vi "ArmPathPlanner.vi"(0 "StartPoint":T5, 1 "EndPoint":T5, 2 "PathPointSpacing (in)":dbl=0.25, 3 "MinArmLength":dbl=44.0, 4 "MaxArmLength":dbl=68.0, 5 "AvoidancePolygon":T4, 7 "MotionProfileGeneratorParameters":T3={"Trajectory Point Interval (ms)"=10, "Maximum Travel Speed (units/s)"=0.0, "Velocity Ramp Time (ms)"=0.0, "Acceleration Ramp Time (ms)"=1.0} {"Acceleration Ramp Time (ms)" min=1.0; "Velocity Ramp Time (ms)" min=1.0; "Maximum Travel Speed (units/s)" min=0.0; "Trajectory Point Interval (ms)" items=["TrajectoryDuration_0ms"=0, "TrajectoryDuration_5ms"=5, "TrajectoryDuration_10ms"=10, "TrajectoryDuration_20ms"=20, "TrajectoryDuration_30ms"=30, "TrajectoryDuration_40ms"=40, "TrajectoryDuration_50ms"=50, "TrajectoryDuration_100ms"=100]}) -> (14 "Path":T6[](array[typedef]), 15 "RotatePath":T1[](array[typedef]) {"Time (ms)" items=["TrajectoryDuration_0ms"=0, "TrajectoryDuration_5ms"=5, "TrajectoryDuration_10ms"=10, "TrajectoryDuration_20ms"=20, "TrajectoryDuration_30ms"=30, "TrajectoryDuration_40ms"=40, "TrajectoryDuration_50ms"=50, "TrajectoryDuration_100ms"=100]}, 16 "ExtendPath":T1[](array[typedef]) {"Time (ms)" items=["TrajectoryDuration_0ms"=0, "TrajectoryDuration_5ms"=5, "TrajectoryDuration_10ms"=10, "TrajectoryDuration_20ms"=20, "TrajectoryDuration_30ms"=30, "TrajectoryDuration_40ms"=40, "TrajectoryDuration_50ms"=50, "TrajectoryDuration_100ms"=100]}, 19 "PathLength (in)":dbl)   [LabVIEW 2017]
uses:
  TypeDefs/ArmCoordinate.ctl
  ArgosLib/Path Planning/TypeDefs/Point2D.ctl
  ArgosLib/Path Planning/TypeDefs/Polygon2D.ctl
  General/MotionProfiling/TypeDefs/MotionProfileGeneratorParams.ctl
  <vilib>/Rock Robotics/WPI/ThirdParty/Phoenix-LabVIEW/Motor Controller/Controls/CTRE_Phoenix_MotorControl_TrajectoryPointTimeDur.ctl
  General/MotionProfiling/TypeDefs/TrajectoryPoint.ctl
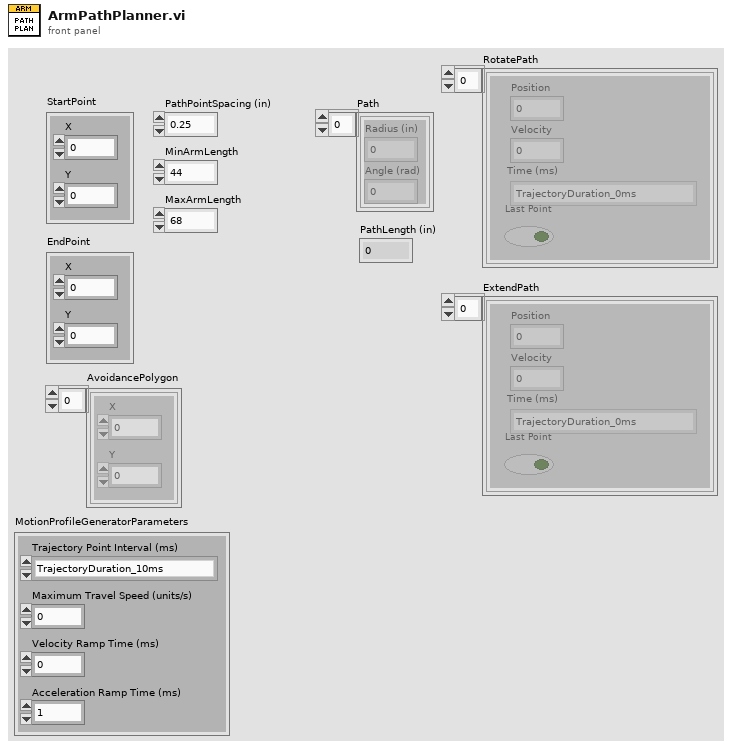
[diagram p1: front panel]
types:
  T1 = typedef "TrajectoryPoint.ctl" = cluster{"Position ":dbl, "Velocity ":dbl, "Time (ms)":T2, "Last Point":bool}
  T2 = typedef "CTRE_Phoenix_MotorControl_TrajectoryPointTimeDur.ctl" = i32
  T3 = typedef "MotionProfileGeneratorParams.ctl" = cluster{"Trajectory Point Interval (ms)":T2, "Maximum Travel Speed (units/s)":dbl, "Velocity Ramp Time (ms)":dbl, "Acceleration Ramp Time (ms)":dbl}
  T4 = typedef "Polygon2D.ctl" = T5[]
  T5 = typedef "Point2D.ctl" = cluster{"X":dbl, "Y":dbl}
  T6 = typedef "ArmCoordinate.ctl" = cluster{"Radius (in)":dbl, "Angle (rad)":dbl}
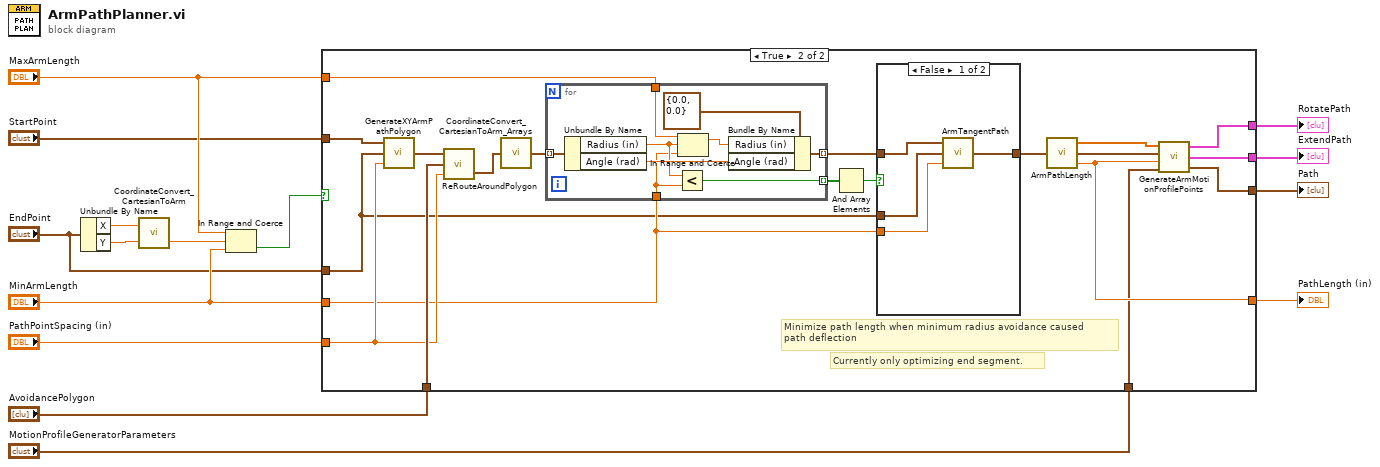
[diagram p0: block diagram]
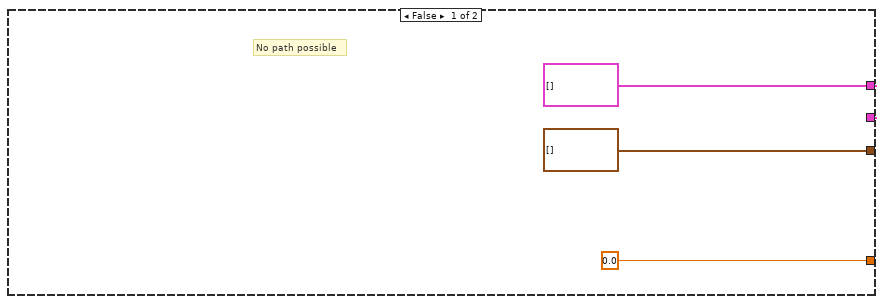
[diagram p2: hidden frame]
diagram:
  n1 = Unbundle By Name("EndPoint") -> ("X"=w8:dbl, "Y"=w7:dbl)
  n2 = call "CoordinateConvert_CartesianToArm.vi"("Y (in)"=w7, "X (in)"=w8) -> ("Radius (in)"=w15:dbl)  [unwired: 1 out]
  n3 = In Range and Coerce(upper limit="MaxArmLength", x=w15, lower limit="MinArmLength") -> (In Range?=w14:bool)  [unwired: 1 out]
  n4 = case shown="True" w14 {
    tunnel: [T6[] [] ("ArmPathOut") w27] -> w9
    tunnel: [0.0 w29] -> w13
    tunnel: "MinArmLength" -> [_ w20]
    tunnel: "MaxArmLength" -> [_ w38]
    tunnel: "PathPointSpacing (in)" -> [_ w33]
    tunnel: "StartPoint" -> [_ w37]
    tunnel: "EndPoint" -> [_ w19]
    tunnel: "AvoidancePolygon" -> [_ w34]
    tunnel: "MotionProfileGeneratorParameters" -> [_ w28]
    tunnel: [w16 w26] -> w2
    tunnel: [w16 w25] -> w1
    frame False {
      w16 = T1[] [] ("ExtendPath")
      # "No path possible"
    }
    frame True {
      # "Currently only optimizing end segment."
      # "Minimize path length when minimum radius avoidance caused\npath deflection"
      n5 = call "GenerateXYArmPathPolygon.vi"("PointSpacing (in)"=w33, "EndPoint"=w19, "StartPoint"=w37) -> ("XYPathPoints"=w35:T5[])
      n6 = call "ReRouteAroundPolygon.vi"("Desired Point Spacing (in)"=w33, "AvoidancePolygon"=w34, "InputPath"=w35) -> ("OutputPath"=w32:T5[])  [unwired: 1 out]
      n7 = call "CoordinateConvert_CartesianToArm_Arrays.vi"("XYPoints"=w32) -> ("ArmCoordinates"=w36:T6[])
      n8 = for {
        tunnel: w38 -> [w52]
        tunnel: w20 -> [w45]
        tunnel: w36 -> [w51] mode=indexing
        tunnel: [w47] -> w22 mode=indexing
        tunnel: [w44] -> w24 mode=indexing
        n9 = Unbundle By Name(w51) -> ("Radius (in)"=w46:dbl, "Angle (rad)"=w50:dbl)
        n10 = Less?(x=w46, y=w45) -> (x < y?=w44:bool)
        n11 = In Range and Coerce(upper limit=w52, x=w46, lower limit=w45) -> (coerced(x)=w49:dbl)  [unwired: 1 out]
        n12 = Bundle By Name(cluster=T6 {"Radius (in)"=0.0, "Angle (rad)"=0.0} ("Point"), "Radius (in)"=w49, "Angle (rad)"=w50) -> (w47:T6)
      }
      n13 = And Array Elements(Boolean array=w24) -> (logical AND=w23:bool)
      n14 = case shown="False" w23 {
        tunnel: w22 -> [w42 w43]
        tunnel: [w39 w43] -> w21
        tunnel: w20 -> [w40 _]
        tunnel: w19 -> [w41 _]
        frame False {
          n15 = call "ArmTangentPath.vi"("Radius"=w40, "EndPoint"=w41, "PathIn"=w42) -> ("PathOut"=w39:T6[])
        }
        frame True {
        }
      }
      n16 = call "ArmPathLength.vi"("ArmPathIn"=w21) -> ("Path Length"=w29:dbl, "ArmPathOut"=w30:T6[], "IndexedPathLength"=w31:dbl[])  [unwired: 2 in]
      n17 = call "GenerateArmMotionProfilePoints.vi"("MotionProfileGeneratorParameters"=w28, "PathDistance"=w29, "ArmPathIn"=w30, "IndexedPathLength"=w31) -> ("ArmPathOut"=w27:T6[], "ExtendPath"=w25:T1[], "RotatePath"=w26:T1[])
    }
  }
  "PathLength (in)" <- w13
  "Path" <- w9
  "RotatePath" <- w2
  "ExtendPath" <- w1
